vi "xnet_canopen_get_status.vi"(8 "error in (no error)":errorcluster, 11 "xnet_co_handle_in":u64) -> (0 "error out":errorcluster, 2 "CANOpen Status":T1 {"NMT State" items=["Unknown"=-1, "Initializing"=0, "Pre-Operational"=127, "Operational"=5, "Stopped"=4, "?"=255]; "can_error_status" format="%.0x"}, 3 "xnet_co_handle":u64)   [LabVIEW 2023, in "xnet_canopen.lvlib"]
uses:
  xnet_canopen.lvlib
  <vilib>/Utility/error.llb/Error Cluster From Error Code.vi
  typedef/canopen status.ctl
  typedef/Runtime State.ctl
  typedef/NMT State.ctl
  typedef/canopen status formatted.ctl
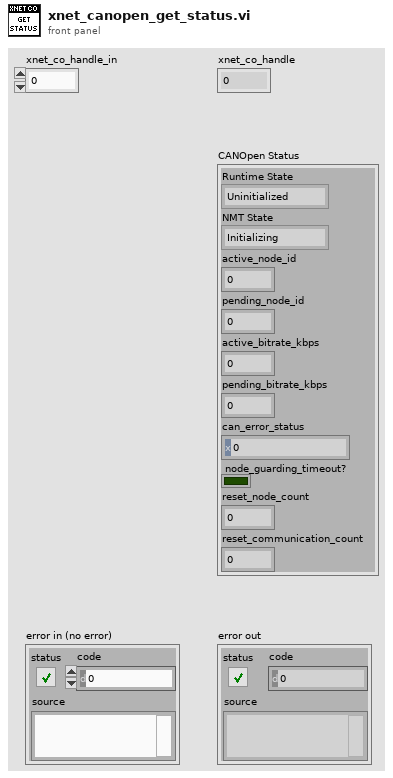
[diagram p1: front panel]
types:
  T1 = typedef "xnet_canopen.lvlib/canopen status formatted.ctl" = cluster{"Runtime State":T2, "NMT State":T3, "active_node_id":u32, "pending_node_id":u32, "active_bitrate_kbps":u32, "pending_bitrate_kbps":u32, "can_error_status":u32, "node_guarding_timeout?":bool, "reset_node_count":u32, "reset_communication_count":u32}
  T2 = typedef "xnet_canopen.lvlib/Runtime State.ctl" = enum16{"Uninitialized", "Stopped", "Running", "Failed", "?"}
  T3 = typedef "xnet_canopen.lvlib/NMT State.ctl" = i32
  T4 = typedef "xnet_canopen.lvlib/canopen status.ctl" = cluster{"runtime_state":u32, "nmt_state":u32, "active_node_id":u32, "pending_node_id":u32, "active_bitrate_kbps":u32, "pending_bitrate_kbps":u32, "can_error_status":u32, "node_guarding_timeout":u32, "reset_node_count":u32, "reset_communication_count":u32}
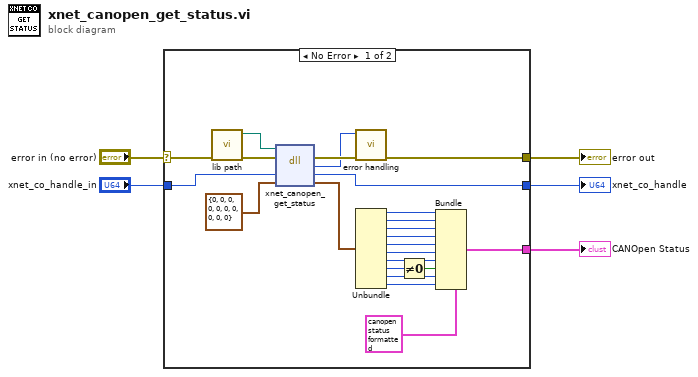
[diagram p0: block diagram]
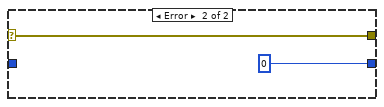
[diagram p2: hidden frame]
diagram:
  n1 = case shown="No Error" "error in (no error)" {
    selector: "error in (no error)" -> [w26 w29]
    tunnel: [w24 w29] -> w4
    tunnel: [w22 u64 0 ("phandle")] -> w3
    tunnel: "xnet_co_handle_in" -> [w21 _]
    tunnel: [w6 _] -> w1
    frame No Error {
      n2 = call "lib path.vi"() -> ("lib path"=w27:path)  [unwired: 11 in]
      n3 = dll-call lib="?" fn="xnet_canopen_get_status"(path in=w27, error in=w26, "handle"=w21, "status"=T4 {"runtime_state"=0, "nmt_state"=0, "active_node_id"=0, "pending_node_id"=0, "active_bitrate_kbps"=0, "pending_bitrate_kbps"=0, "can_error_status"=0, "node_guarding_timeout"=0, "reset_node_count"=0, "reset_communication_count"=0} ("CANOpen Status")) -> (error out=w25:errorcluster, "return type"=w23:i32, "handle"=w22:u64, "status"=w19:T4)  [unwired: 1 in, 1 out]
      n4 = call "error handling.vi"("error in (no error)"=w25, "return val"=w23) -> ("error out"=w24:errorcluster)  [unwired: 9 in]
      n5 = Unbundle(w19) -> ("runtime_state"=w17:u32, "nmt_state"=w16:u32, "active_node_id"=w15:u32, "pending_node_id"=w14:u32, "active_bitrate_kbps"=w13:u32, "pending_bitrate_kbps"=w12:u32, "can_error_status"=w11:u32, "node_guarding_timeout"=w10:u32, "reset_node_count"=w9:u32, "reset_communication_count"=w8:u32)
      n6 = Not Equal To 0?(x=w10) -> (x != 0?=w7:bool)
      n7 = Bundle(cluster=T1 {"Runtime State"=enum."Uninitialized", "NMT State"=0, "active_node_id"=0, "pending_node_id"=0, "active_bitrate_kbps"=0, "pending_bitrate_kbps"=0, "can_error_status"=0, "node_guarding_timeout?"=FALSE, "reset_node_count"=0, "reset_communication_count"=0} ("CANOpen Status Formatted"), "Runtime State"=w17, "NMT State"=w16, "active_node_id"=w15, "pending_node_id"=w14, "active_bitrate_kbps"=w13, "pending_bitrate_kbps"=w12, "can_error_status"=w11, "node_guarding_timeout?"=w7, "reset_node_count"=w9, "reset_communication_count"=w8) -> (w6:T1)
    }
    frame Error {
    }
  }
  "error out" <- w4
  "xnet_co_handle" <- w3
  "CANOpen Status" <- w1
